vi "term_connect_wire.vi"() -> ()   [LabVIEW 2014]
panel:
  out "error out":errorcluster
  out "reference out":refnum<vi>
  in  "Auto Route? (F)":bool
  in  "Wiring Specs":string[][](array[string])
  in  "Auto Wire? (T)":bool
  in  "Wire Source":refnum<vi>
  in  "error in (no error)":errorcluster
  in  "reference":refnum<vi>
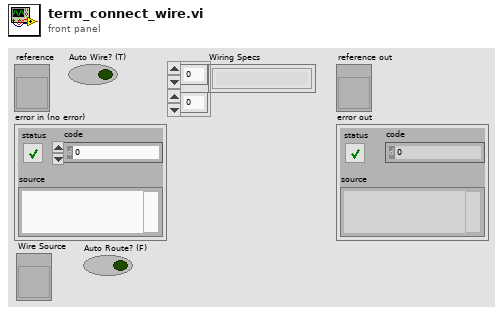
[diagram p1: front panel]
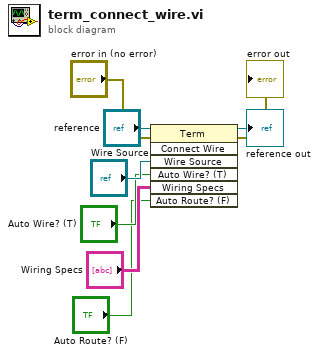
[diagram p0: block diagram]
diagram:
  n1 = invoke class="Term" method="Connect Wire"(reference="reference", error in="error in (no error)", "Wire Source"="Wire Source", "Auto Wire? (T)"="Auto Wire? (T)", "Wiring Specs"="Wiring Specs", "Auto Route? (F)"="Auto Route? (F)") -> (reference out=→"reference out":refnum<vi>, error out=→"error out":errorcluster)  [unwired: 1 in, 5 out]
